vi "VIH Utility - UI - Highlight Text in Control.vi"(11 "FocusObj":refnum<vi>) -> (0 "OK":bool)   [LabVIEW 2014]
doc: "::: VI Helpeks :::\nCopyright (c) 2000-2026 Konstantin Shifershteyn. All rights reserved."
panel:
  # "VI Helpeks\nCopyright (c) 2012-2026 Konstantin Shifershteyn"
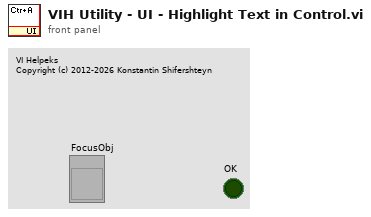
[diagram p1: front panel]
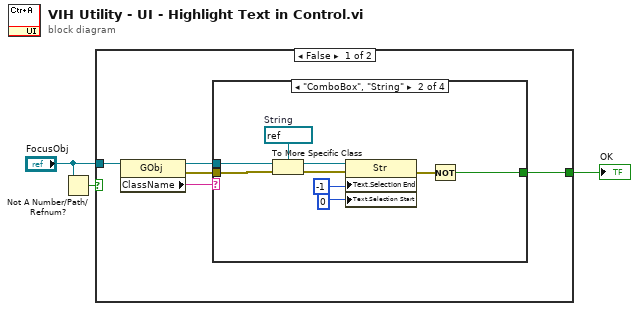
[diagram p0: block diagram]
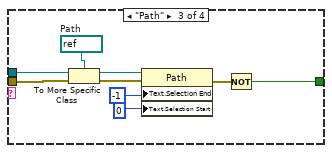
[diagram p3: hidden frame]
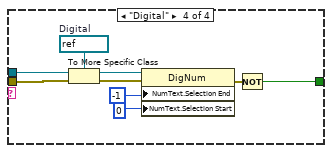
[diagram p4: hidden frame]
diagram:
  n1 = Not A Number/Path/Refnum?(number/path/refnum="FocusObj") -> (NaN/Path/Refnum?=w2:bool)
  n2 = case shown="False" w2 {
    tunnel: [w8 _] -> w3
    tunnel: "FocusObj" -> [w4 _]
    frame False {
      n3 = property class="GObj"(reference=w4) -> (reference out=w6:refnum<vi>, error out=w7:errorcluster, "ClassName"=w5:string)  [unwired: 1 in]
      n4 = case shown="\"ComboBox\", \"String\"" w5 {
        tunnel: w6 -> [_ w11 w20 w29]
        tunnel: w7 -> [_ w10 w19 w28]
        tunnel: [_ w9 w18 w27] -> w8
        frame Default {
        }
        frame "ComboBox", "String" {
          w17 = refnum<vi> refnum  # String
          n5 = To More Specific Class(target class=w17, reference=w11, error in=w10) -> (specific class reference=w16:refnum<vi>, error out=w15:errorcluster)
          n6 = property class="Str"(reference=w16, error in=w15, "Text.Selection End"=-1, "Text.Selection Start"=0) -> (error out=w12:errorcluster)  [unwired: 1 out]
          n7 = Not(x=w12) -> (.not. x?=w9:bool)
        }
        frame "Path" {
          w26 = refnum<vi> refnum  # Path
          n8 = To More Specific Class(target class=w26, reference=w20, error in=w19) -> (specific class reference=w25:refnum<vi>, error out=w24:errorcluster)
          n9 = property class="Path"(reference=w25, error in=w24, "Text.Selection End"=-1, "Text.Selection Start"=0) -> (error out=w21:errorcluster)  [unwired: 1 out]
          n10 = Not(x=w21) -> (.not. x?=w18:bool)
        }
        frame "Digital" {
          w35 = refnum<vi> refnum  # Digital
          n11 = To More Specific Class(target class=w35, reference=w29, error in=w28) -> (specific class reference=w34:refnum<vi>, error out=w33:errorcluster)
          n12 = property class="DigNum"(reference=w34, error in=w33, "NumText.Selection End"=-1, "NumText.Selection Start"=0) -> (error out=w30:errorcluster)  [unwired: 1 out]
          n13 = Not(x=w30) -> (.not. x?=w27:bool)
        }
      }
    }
    frame True {
    }
  }
  "OK" <- w3
